vi "Migrate - Needs Migration.vi"(8 "error in (no error)":errorcluster, 11 "Data Folder":path) -> (0 "error out":errorcluster, 3 "needs migration?":bool)   [LabVIEW 2024]
doc: "TRUE when the data folder holds version-1 data: Projects.ini exists and has no [_Meta] Schema Version = 2. FALSE when Projects.ini is missing (nothing to migrate) or is already version 2.\n\nGenerated by: Claude"
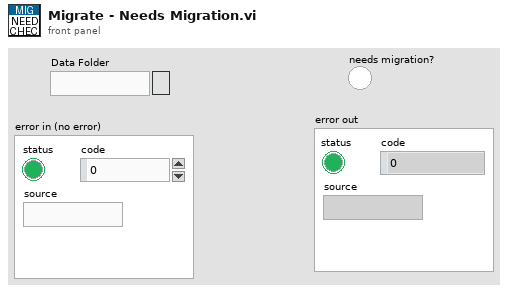
[diagram p1: front panel]
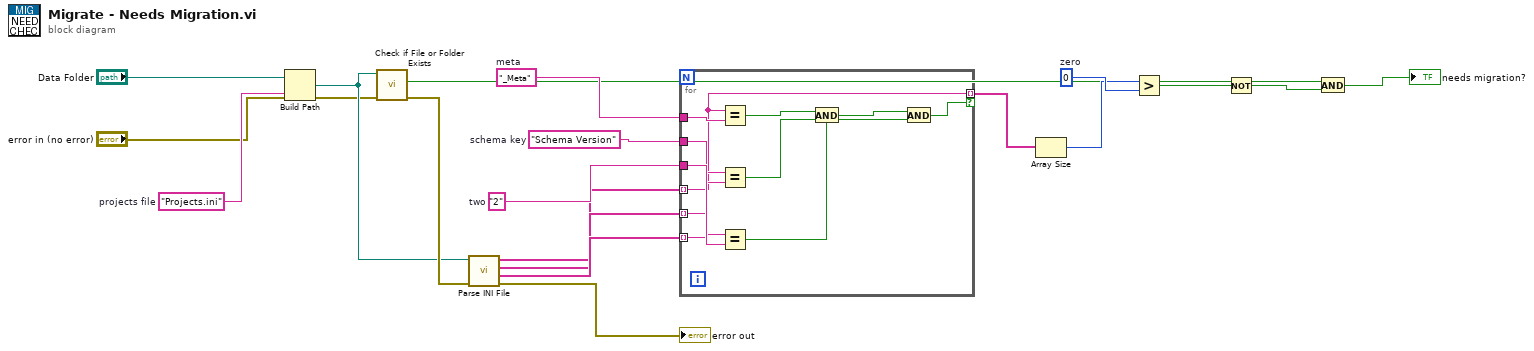
[diagram p0: block diagram]
diagram:
  w16 = 0  # zero
  w13 = "2"  # two
  w12 = "Schema Version"  # schema key
  w11 = "_Meta"  # meta
  w3 = "Projects.ini"  # projects file
  n1 = Build Path(base path="Data Folder", name or relative path=w3) -> (appended path=w4:path)
  n2 = call <vilib>:"Check if File or Folder Exists.vi"("error in (no error)"="error in (no error)", "path"=w4) -> ("error out"=w5:errorcluster, "file or folder exists?"=w6:bool)  [unwired: 7 in, 1 out]
  n3 = call "Parse INI File.vi"("error in (no error)"=w5, "File Path"=w4) -> ("error out"=→"error out":errorcluster, "Values"=w9:string[], "Keys"=w8:string[], "Sections"=w7:string[])  [unwired: 6 in]
  n4 = for {
    tunnel: w11 -> [w23]
    tunnel: w12 -> [w24]
    tunnel: w13 -> [w25]
    tunnel: w7 -> [w20] mode=indexing
    tunnel: w8 -> [w21] mode=indexing
    tunnel: w9 -> [w22] mode=indexing
    tunnel: [w20] -> w14 mode=indexing if=w30
    n5 = Equal?(x=w20, y=w23) -> (x = y?=w26:bool)
    n6 = Equal?(x=w21, y=w24) -> (x = y?=w27:bool)
    n7 = Equal?(x=w22, y=w25) -> (x = y?=w28:bool)
    n8 = And(x=w26, y=w27) -> (x .and. y?=w29:bool)
    n9 = And(x=w29, y=w28) -> (x .and. y?=w30:bool)
  }
  n10 = Array Size(array=w14) -> (size(s)=w15:i32)
  n11 = Greater?(x=w15, y=w16) -> (0:w17:bool)
  n12 = Not(x=w17) -> (.not. x?=w18:bool)
  n13 = And(x=w6, y=w18) -> (x .and. y?=→"needs migration?":bool)
